vi "激光控制状态机.vi"(6 "写入data":u16, 7 "标刻内容":T1, 8 "错误输入（无错误）":errorcluster, 9 "debug项目路径":path, 10 "EZCAD模板路径":path, 11 "激光控制":T2) -> (0 "错误输出":errorcluster, 2 "IsMarking":bool, 3 "LoadEzdFile_resultstatus":i32, 4 "WritePort 2":i32, 5 "读取数据":cluster{"ReadPort":i32, "读取data":u16})   [LabVIEW 2021]
uses:
  C:/Users/skate/OneDrive/0_Github_App_/lazer_cad/lazer_cad_demo/LazerClassLibrary/bin/x86/Debug/LazerClassLibrary.dll
  LazerClassLibrary/bin/x86/Debug/LazerClassLibrary.dll
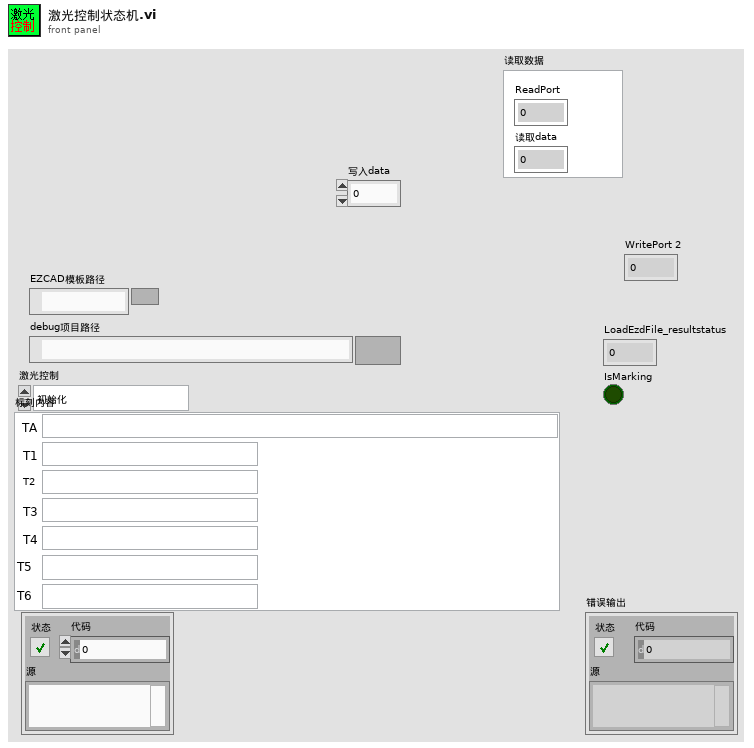
[diagram p1: front panel]
types:
  T1 = typedef "标刻内容.ctl" = cluster{"T1":string, "T2":string, "T3":string, "T4":string, "TA":string, "T5":string, "T6":string}
  T2 = typedef "激光控制.ctl" = enum16{"初始化", "等待", "初始化激光", "加载模板", "替换字符", "启动刻码", "检测刻码完成", "读取端口", "写入端口", "停止标刻", "关闭调用", "释放", "退出"}
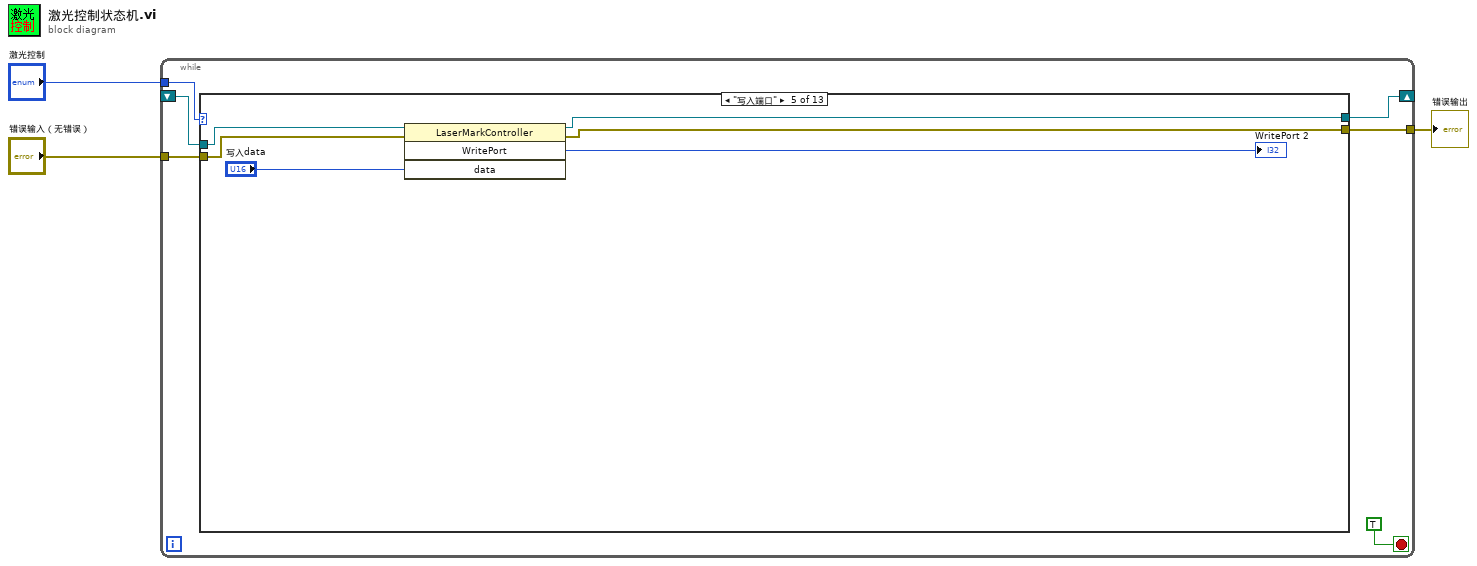
[diagram p0: block diagram]
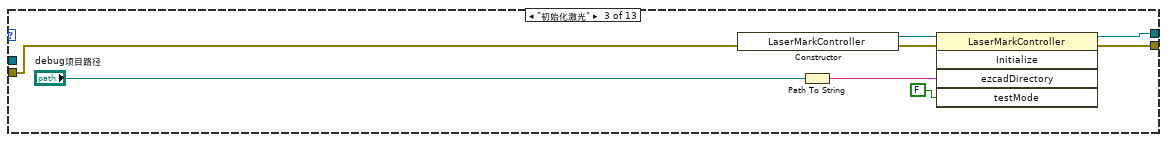
[diagram p4: hidden frame]
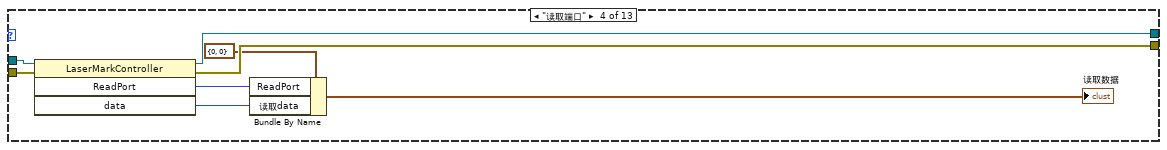
[diagram p5: hidden frame]
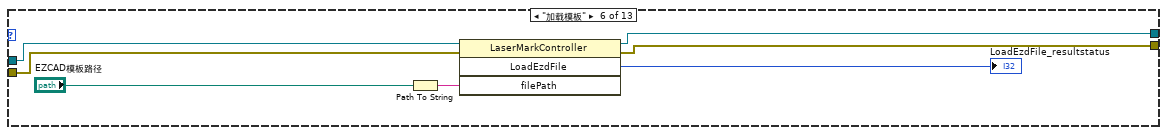
[diagram p6: hidden frame]
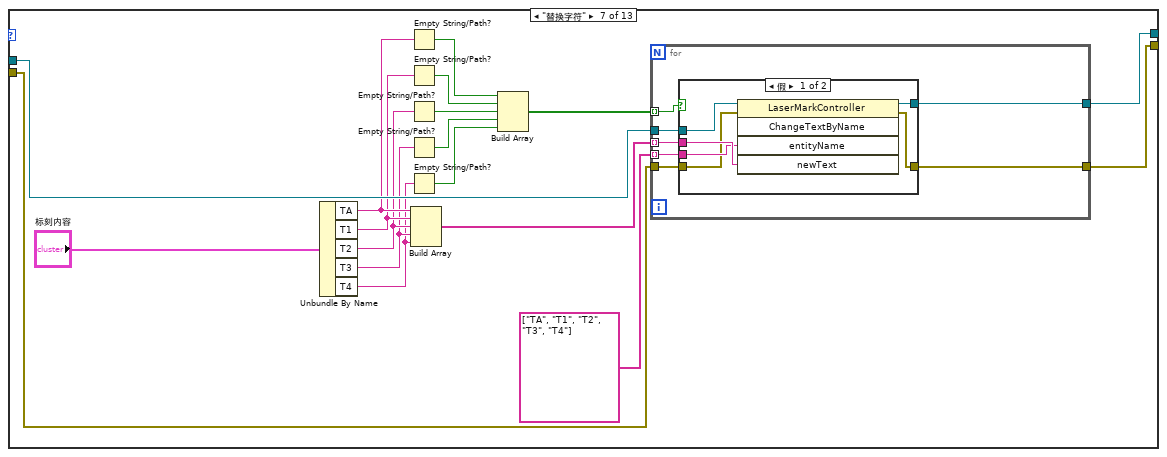
[diagram p7: hidden frame]
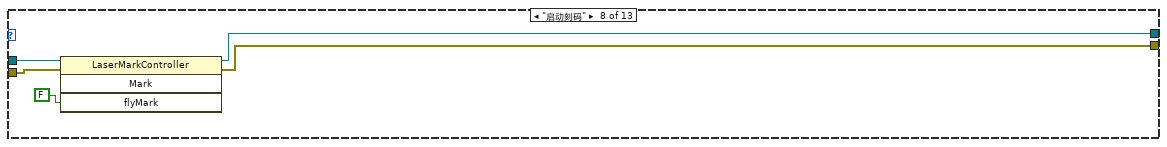
[diagram p9: hidden frame]
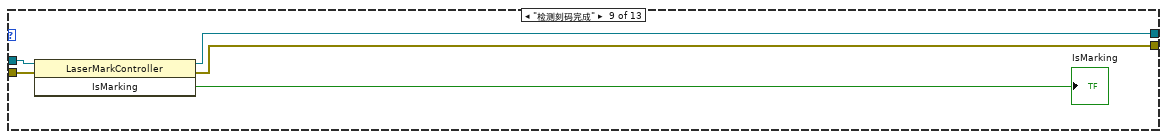
[diagram p10: hidden frame]
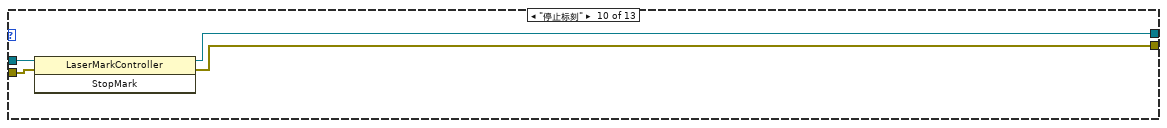
[diagram p11: hidden frame]
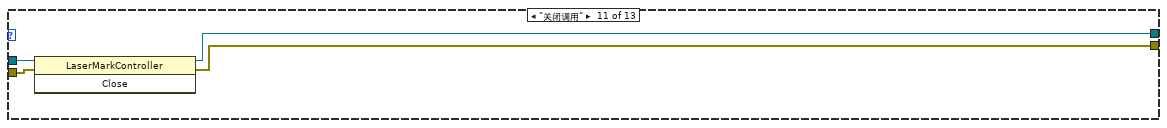
[diagram p12: hidden frame]
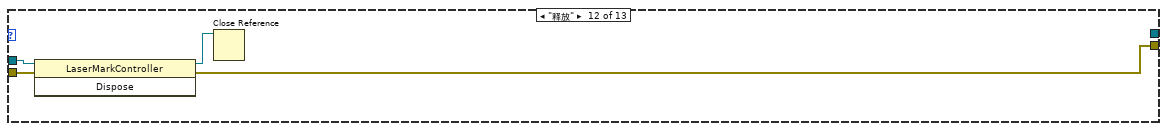
[diagram p13: hidden frame]
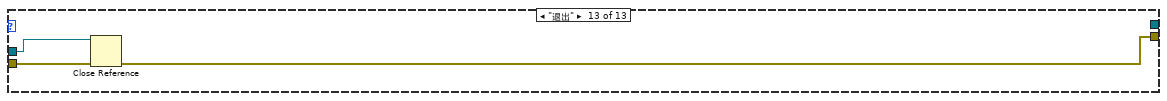
[diagram p14: hidden frame]
diagram:
  n1 = while {
    tunnel: "激光控制" -> [w8]
    tunnel: "错误输入（无错误）" -> [w7]
    tunnel: [w6] -> w1
    shift-right: [w5] -> _
    shift-left: _ -> [w4]
    stop <- TRUE stop-if-true
    n2 = case shown="\"写入端口\"" w8 {
      tunnel: w7 -> [w10 w12 w21 w28 w34 w38 w43 w78 w82 w87 w90 w96 w99]
      tunnel: [w10 w12 w19 w26 w32 w37 w44 w77 w81 w86 w91 w95 w98] -> w6
      tunnel: [w11 w13 w18 w27 w33 w39 w52 w79 w84 w88 w92 _ _] -> w5
      tunnel: w4 -> [w11 w13 _ w29 w35 w42 w60 w80 w85 w89 w93 w97 w100]
      frame "初始化" {
      }
      frame "等待", Default {
      }
      frame "初始化激光" {
        n3 = constructor class="LaserMarkController"(error in=w21) -> (reference out=w14:refnum<k24>, error out=w20:errorcluster)  [unwired: 2 in, 1 out]
        n4 = Path To String(path="debug项目路径") -> (string=w17:string)
        n5 = invoke class="LaserMarkController" method="Initialize"(reference=w14, error in=w20, "ezcadDirectory"=w17, "testMode"=FALSE) -> (reference out=w18:refnum<k24>, error out=w19:errorcluster)  [unwired: 1 in, 3 out]
      }
      frame "读取端口" {
        n6 = invoke class="LaserMarkController" method="ReadPort"(reference=w29, error in=w28) -> (reference out=w27:refnum<k24>, error out=w26:errorcluster, "ReadPort"=w24:i32, "data"=w23:u16)  [unwired: 2 in]
        n7 = Bundle By Name(cluster=cluster{"ReadPort":i32, "读取data":u16} {"ReadPort"=0, "读取data"=0} ("读取数据"), "ReadPort"=w24, "读取data"=w23) -> (→"读取数据":cluster{"ReadPort":i32, "读取data":u16})
      }
      frame "写入端口" {
        n8 = invoke class="LaserMarkController" method="WritePort"(reference=w35, error in=w34, "data"="写入data") -> (reference out=w33:refnum<k24>, error out=w32:errorcluster, "WritePort"=→"WritePort 2":i32)  [unwired: 1 in, 1 out]
      }
      frame "加载模板" {
        n9 = Path To String(path="EZCAD模板路径") -> (string=w40:string)
        n10 = invoke class="LaserMarkController" method="LoadEzdFile"(reference=w42, error in=w38, "filePath"=w40) -> (reference out=w39:refnum<k24>, error out=w37:errorcluster, "LoadEzdFile"=→"LoadEzdFile_resultstatus":i32)  [unwired: 1 in, 1 out]
      }
      frame "替换字符" {
        n11 = Unbundle By Name("标刻内容") -> ("TA"=w51:string, "T1"=w50:string, "T2"=w49:string, "T3"=w48:string, "T4"=w47:string)
        n12 = Empty String/Path?(string/path=w51) -> (empty?=w58:bool)
        n13 = Empty String/Path?(string/path=w50) -> (empty?=w57:bool)
        n14 = Empty String/Path?(string/path=w49) -> (empty?=w56:bool)
        n15 = Empty String/Path?(string/path=w48) -> (empty?=w55:bool)
        n16 = Empty String/Path?(string/path=w47) -> (empty?=w54:bool)
        n17 = Build Array(w51, w50, w49, w48, w47) -> (w46:string[])
        n18 = Build Array(w58, w57, w56, w55, w54) -> (w53:bool[])
        n19 = for {
          tunnel: w60 -> [w67]
          tunnel: w53 -> [w65] mode=indexing
          tunnel: [w66] -> w52
          tunnel: w46 -> [w64] mode=indexing
          tunnel: string[] ["TA", "T1", "T2", "T3", "T4"] ("T1") -> [w63] mode=indexing
          tunnel: [w62] -> w44
          tunnel: w43 -> [w61]
          n20 = case shown="假" w65 {
            tunnel: w67 -> [w73 w75]
            tunnel: [w72 w75] -> w66
            tunnel: w64 -> [w71 _]
            tunnel: w63 -> [w70 _]
            tunnel: [w69 w74] -> w62
            tunnel: w61 -> [w68 w74]
            frame False {
              n21 = invoke class="LaserMarkController" method="ChangeTextByName"(reference=w73, error in=w68, "entityName"=w70, "newText"=w71) -> (reference out=w72:refnum<k24>, error out=w69:errorcluster)  [unwired: 1 in, 3 out]
            }
            frame True {
            }
          }
        }
      }
      frame "启动刻码" {
        n22 = invoke class="LaserMarkController" method="Mark"(reference=w80, error in=w78, "flyMark"=FALSE) -> (reference out=w79:refnum<k24>, error out=w77:errorcluster)  [unwired: 1 in, 2 out]
      }
      frame "检测刻码完成" {
        n23 = invoke class="LaserMarkController" method="IsMarking"(reference=w85, error in=w82) -> (reference out=w84:refnum<k24>, error out=w81:errorcluster, "IsMarking"=→"IsMarking":bool)  [unwired: 1 in]
      }
      frame "停止标刻" {
        n24 = invoke class="LaserMarkController" method="StopMark"(reference=w89, error in=w87) -> (reference out=w88:refnum<k24>, error out=w86:errorcluster)  [unwired: 1 in, 1 out]
      }
      frame "关闭调用" {
        n25 = invoke class="LaserMarkController" method="Close"(reference=w93, error in=w90) -> (reference out=w92:refnum<k24>, error out=w91:errorcluster)  [unwired: 1 in, 1 out]
      }
      frame "释放" {
        n26 = invoke class="LaserMarkController" method="Dispose"(reference=w97, error in=w96) -> (reference out=w94:refnum<k24>, error out=w95:errorcluster)  [unwired: 1 in, 1 out]
        n27 = Close Reference(reference=w94) -> ()  [unwired: 1 in, 1 out]
      }
      frame "退出" {
        n28 = Close Reference(reference=w100, error in (no error)=w99) -> (error out=w98:errorcluster)
      }
    }
  }
  "错误输出" <- w1
